vi "file reader.vi"() -> ()   [LabVIEW 2012]
panel:
  in  "Plots":enum32{"Real", "Imaginary", "Complex Plane"}(tab)
  out "Real":cluster{"X":dbl[], "Y Real":dbl[]}[](graph)
  out "Imaginary":cluster{"X":dbl[], "Y Real":dbl[]}[](graph)
  out "Complex Plane":cluster{"Y Real":dbl[], "Y Imaginary":dbl[]}[](graph)
  in  "Path":path
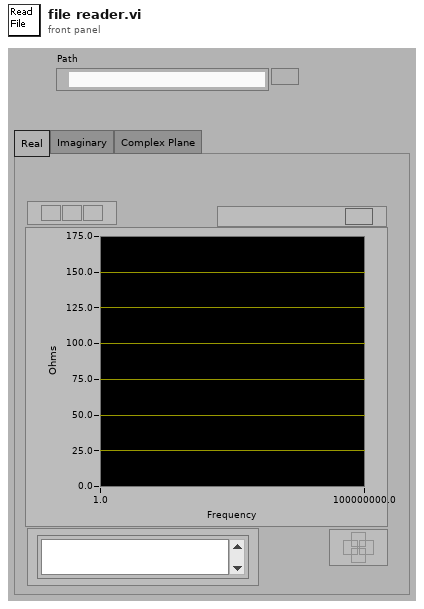
[diagram p1: front panel]
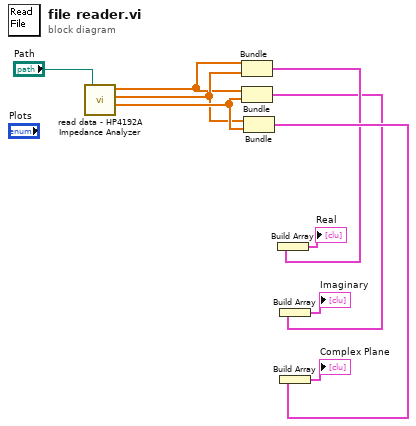
[diagram p0: block diagram]
diagram:
  n1 = call "read data - HP4192A Impedance Analyzer.vi"("file path (dialog if empty)"="Path") -> ("Hz"=w1:dbl[], "R"=w2:dbl[], "X"=w3:dbl[])  [unwired: 1 out]
  n2 = Bundle("Hz"=w1, "R"=w2) -> (w6:cluster{"Hz":dbl[], "R":dbl[]})  [unwired: 1 in]
  n3 = Bundle("Hz"=w1, "X"=w3) -> (w5:cluster{"Hz":dbl[], "X":dbl[]})  [unwired: 1 in]
  n4 = Bundle("R"=w2, "X"=w3) -> (w7:cluster{"R":dbl[], "X":dbl[]})  [unwired: 1 in]
  n5 = Build Array(w6) -> (→"Real":cluster{"Hz":dbl[], "R":dbl[]}[])
  n6 = Build Array(w5) -> (→"Imaginary":cluster{"Hz":dbl[], "X":dbl[]}[])
  n7 = Build Array(w7) -> (→"Complex Plane":cluster{"R":dbl[], "X":dbl[]}[])
